vi "Measurement UI.vi"() -> ()   [LabVIEW 2025, in "Automotive Vision UI.lvlib"]
uses:
  Automotive Vision UI.lvlib
  <vilib>/vision/Image Controls.llb/IMAQ Image.ctl
  <vilib>/gRPC/LabVIEW gRPC Library/Shared/grpcId.ctl
  <vilib>/gRPC/LabVIEW gRPC Library/grpc-lvsupport-release.lvlib
  Automotive-Vision-OOBService_client/Automotive-Vision-OOBService_client.lvlib
  Automotive-Vision-OOBService_client/RPC Messages/hwval_ExportRequest.ctl
  Automotive-Vision-OOBService_client/RPC Messages/hwval_BoolRequest.ctl
  Automotive-Vision-OOBService_client/RPC Messages/hwval_ExportFileType.ctl
  Automotive-Vision-OOBService_client/RPC Messages/hwval_ExportTypeRequest.ctl
  auto vision config.ctl
  register.ctl
panel:
  out "COUNT LENGTH":u64
  out "REGISTERS":string[][](table)
  out "FRAME COUNT BYTES":u32[](array[numeric]) format="%02x"
  in  "config":string="{\n  \"RIO Device\":\"PXI1Slot4\",\n  \"Serial Channel\":\"SI0, SI1, SI2, SI3\",\n  \"SERDES Script\":\"C:\\\\dev\\\\ttashjia\\\\GSE\\\\Host\\\\Scripts\\\\DS90UB954\\\\Acq\\\\Loopback.py\",\n  \"POC Source\":0,\n  \"CSI-2 Data Source\":1,\n  \"Lane Count\":4,\n  \"Reference Clock\":25000000,\n  \"Image Data Type\":44,\n  \"Interpretation\":1,\n  \"Pattern\":3,\n  \"Algorithm\":0,\n  \"Virtual Channel\":0,\n  \"Embedded Data\":{\n    \"Pre-embedded Lines\":4,\n    \"Pre-embedded Line Length\":1920,\n    \"Post-embedded Lines\":2,\n    \"Post-embedded Line Length\":1920,\n    \"Frame Count\":{\"Line\":0,\"Offset\":2,\"Byte Count\":4}\n  },\n  \"Registers\":[\n    {\n      \"Name\":\"Temp0\",\n      \"Device\":97,\n      \"Address\":27,\n      \"Min\":0,\n      \"Max\":16\n    },\n    {\n      \"Name\":\"Temp1\",\n      \"Device\":97,\n      \"Address\":90,\n      \"Min\":0,\n      \"Max\":16\n    }\n  ],\n  \"Log Path\":\"C:\\\\data\"\n}"
  out "WIDTH":u64
  out "HEIGHT":u64
  out "Numeric":i32
  out "error out":errorcluster
  in  "GRPC status":string
  out "OOB gRPC Port":i32
  in  "BITFILE":string="IMAGE RESOLUTION: 800x600 - RAW12"
  out "Available SI Devices":string[][](array[string])
  in  "RIO HANDLER":string
  out "BYTES ACQUIRED":u64 format="%#.6p"
  out "ERROR":bool
  out "IMAGE PIXEL DATA":u32[](array[numeric])
  in  "IMAGE SAVE FORMAT":u32(ring) items=["PNG", "RAW LLP"]
  out "FRAME COUNT":u64
  out "IMAGE DATA":string
  in  "PAUSE":bool
  in  "CAPTURE":bool
  in  "PATH TO IMAGE CAPTURE":path=path "0"
  in  "SERIAL CHANNEL":string="SI1"
  out "SOURCE RATE (fps)":dbl
  out "STATE MESSAGE":string
  out "POC CURRENT (A)":dbl
  out "POC VOLTAGE (V)":dbl
  out "ACQ. DURATION (s)":dbl
  out "ACQ. IN PROGRESS":bool
  out "DISPLAY":T1(plugin-control)
  # "CONFIGURATION"
  # "Image path parameters"
  # "CONTROL"
  # "MONITOR"
  # "STATUS"
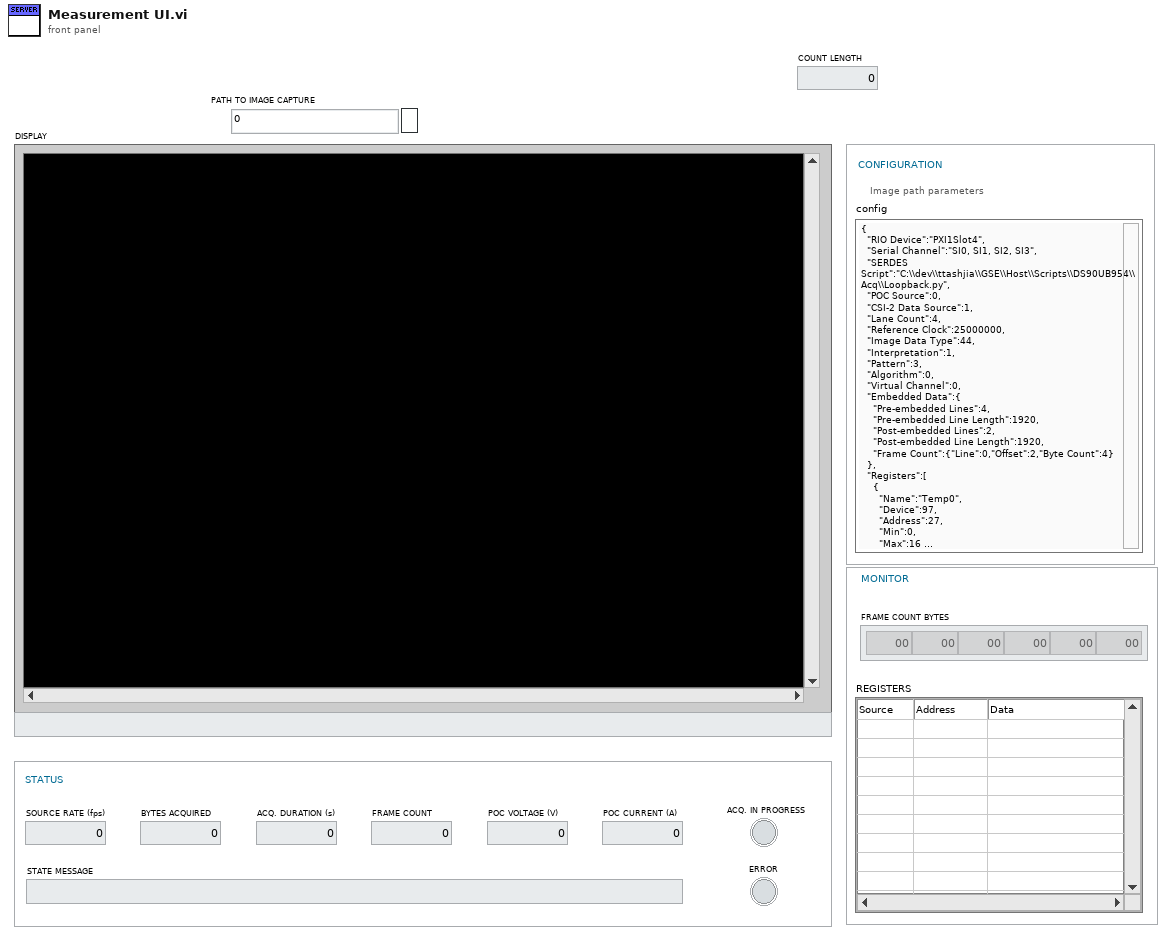
[diagram p1: front panel]
types:
  T1 = typedef "IMAQ Image.ctl" = refnum<image>
  T2 = typedef "Automotive Vision UI.lvlib/auto vision config.ctl" = cluster{"RIO Device":string, "Serial Channel":string, "SERDES Script":string, "POC Source":u32, "CSI-2 Data Source":u32, "Lane Count":u32, "Reference Clock":dbl, "Image Data Type":u32, "Interpretation":u32, "Pattern":u32, "Algorithm":u32, "Virtual Channel":u32, "Embedded Data":cluster{"Pre-embedded Lines":dbl, "Pre-embedded Line Length":dbl, "Post-embedded Lines":dbl, "Post-embedded Line Length":dbl, "Frame Count":cluster{"Line":dbl, "Offset":dbl, "Byte Count":dbl}}, "Registers":T3[], "Log Path":string}
  T3 = typedef "Automotive Vision UI.lvlib/register.ctl" = cluster{"Name":string, "Device":u8, "Address":u16, "Min":u16, "Max":u16}
  T4 = typedef "grpc-lvsupport-release.lvlib/grpcId.ctl" = u64
  T5 = cluster{"pattern":i32, "algorithm":i32, "red gain":dbl, "green gain":dbl, "blue gain":dbl}
  T6 = typedef "Automotive-Vision-OOBService_client.lvlib/hwval_BoolRequest.ctl" = cluster{"BooleanData":bool}
  T7 = typedef "Automotive-Vision-OOBService_client.lvlib/hwval_ExportRequest.ctl" = cluster{"FilePath":string}
  T8 = typedef "Automotive-Vision-OOBService_client.lvlib/hwval_ExportTypeRequest.ctl" = cluster{"FileType":T9}
  T9 = typedef "Automotive-Vision-OOBService_client.lvlib/hwval_ExportFileType.ctl" = enum32{"EXPORT_PNG", "EXPORT_RAW"}
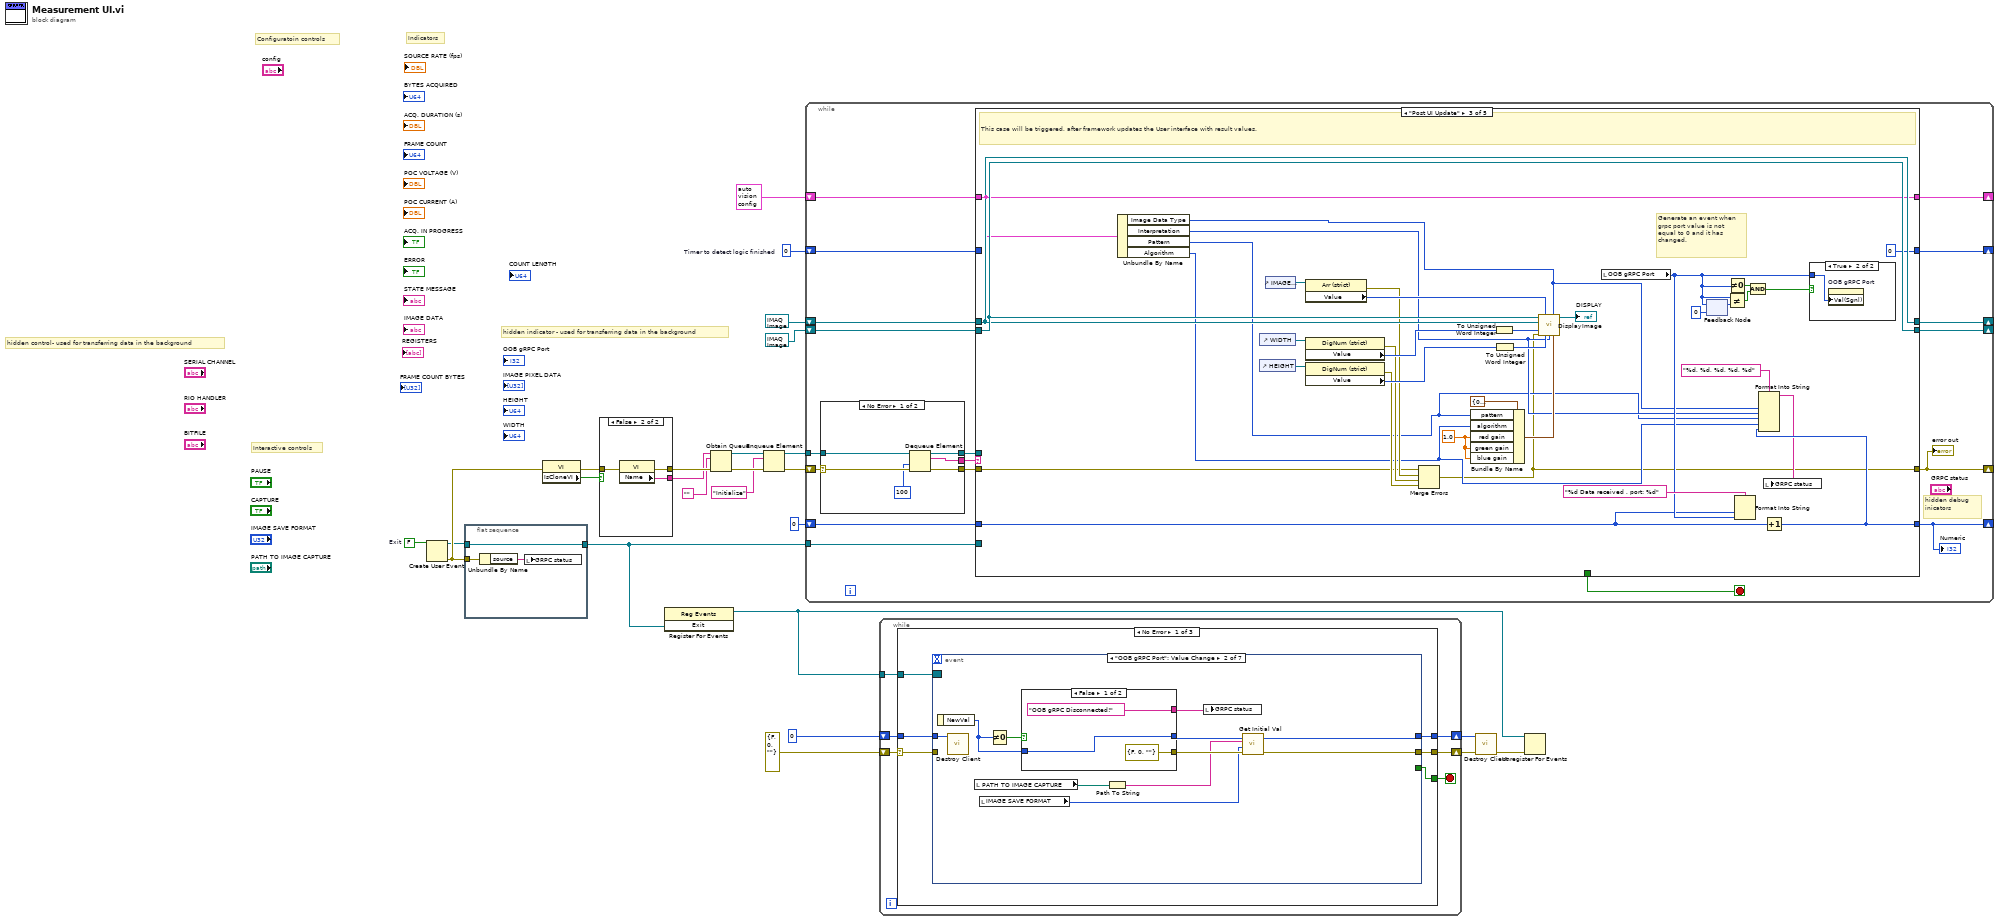
[diagram p0: block diagram]
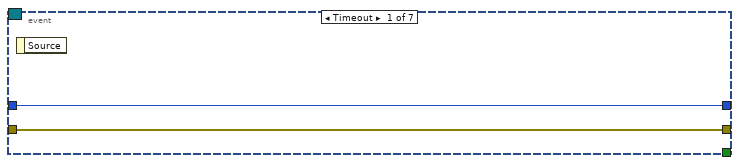
[diagram p2: hidden frame]
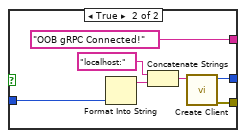
[diagram p3: hidden frame]
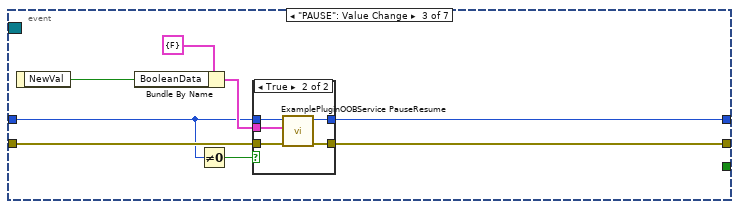
[diagram p4: hidden frame]
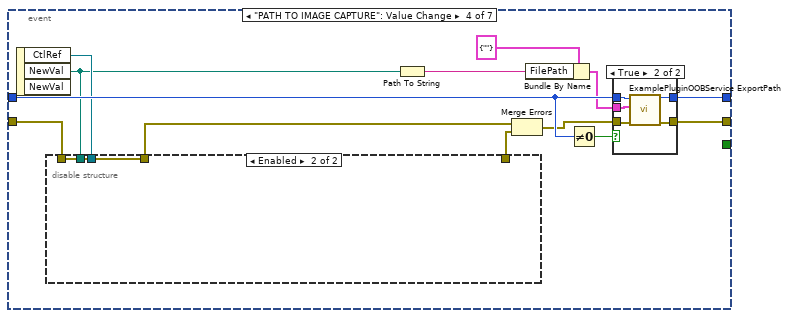
[diagram p6: hidden frame]
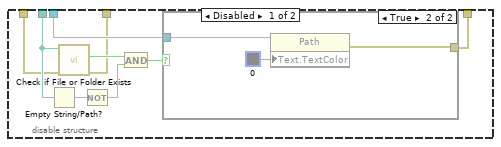
[diagram p7: hidden frame]
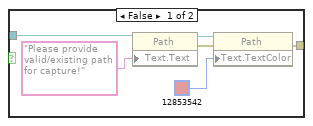
[diagram p8: hidden frame]
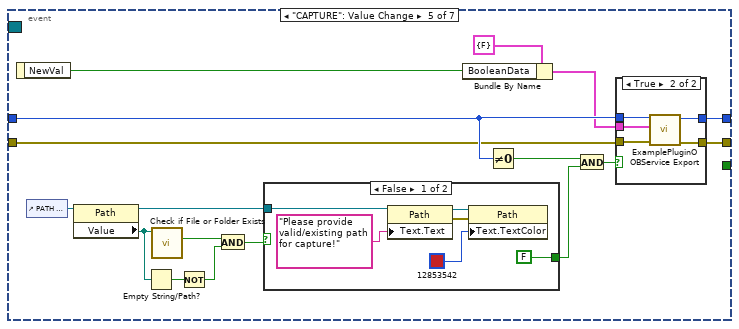
[diagram p10: hidden frame]
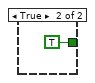
[diagram p11: hidden frame]
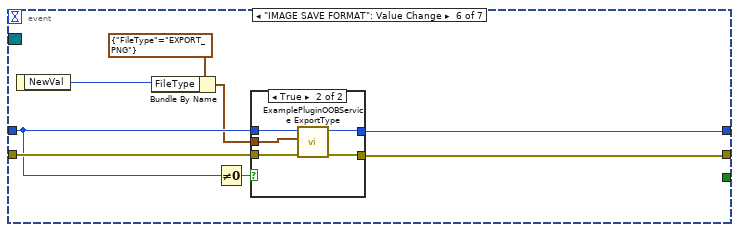
[diagram p13: hidden frame]
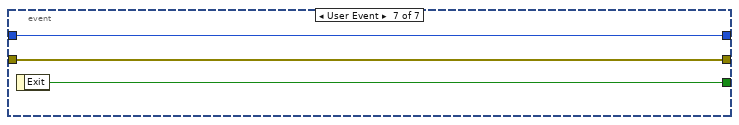
[diagram p15: hidden frame]
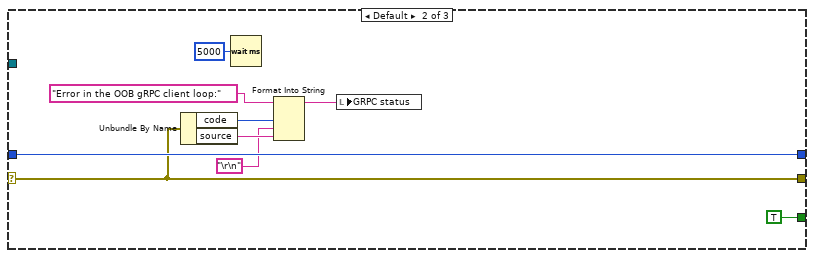
[diagram p16: hidden frame]
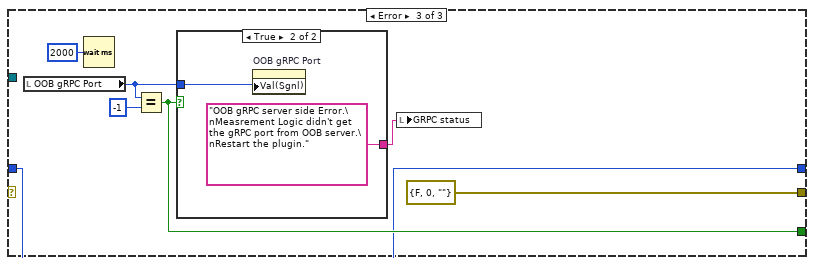
[diagram p17: hidden frame]
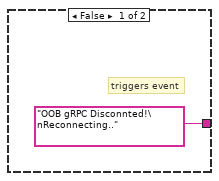
[diagram p18: hidden frame]
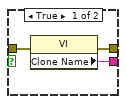
[diagram p19: hidden frame]
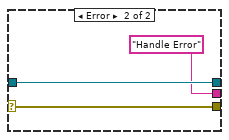
[diagram p20: hidden frame]
diagram:
  w6 = 0  # Timer to detect logic finished
  w15 = FALSE  # Exit
  # "Indicators"
  # "Configuratoin controls"
  # "Interactive controls"
  # "hidden indicator - used for transferring data in the background"
  # "hidden control- used for transferring data in the background"
  n1 = Create User Event(user event datatype=w15) -> (user event=w2:refnum<user-event>, error out=w8:errorcluster)  [unwired: 1 in]
  n2 = flat-sequence {
    tunnel: [w28] -> w9
    tunnel: w2 -> [w28]
    tunnel: w8 -> [w27]
    frame #0 {
      n3 = Unbundle By Name(w27) -> ("source"=w26:string)
      n4 = local write "GRPC status"(w26) -> ()
    }
  }
  n5 = property on="Property Node" class="VI"(error in=w8) -> (error out=w16:errorcluster, "IsCloneVI"=w17:bool)  [unwired: 1 in, 1 out]
  n6 = case shown="False" w17 {
    tunnel: [w31 w34] -> w25
    tunnel: [w30 w33] -> w24
    tunnel: w16 -> [w29 w32]
    frame True {
      n7 = property on="Property Node" class="VI"(error in=w29) -> (error out=w31:errorcluster, "Clone Name"=w30:string)  [unwired: 1 in, 1 out]
    }
    frame False {
      n8 = property on="Property Node" class="VI"(error in=w32) -> (error out=w34:errorcluster, "Name"=w33:string)  [unwired: 1 in, 1 out]
    }
  }
  n9 = register-events(w9) -> (reference out=w14:refnum<event-registration>)  [unwired: 2 in, 1 out]
  n10 = Obtain Queue(name (unnamed)=w24, element data type="" ("Empty String Constant"), error in (no error)=w25) -> (queue out=w21:refnum<queue>, error out=w23:errorcluster)  [unwired: 2 in, 1 out]
  n11 = Enqueue Element(queue=w21, element="Initialize", error in (no error)=w23) -> (queue out=w20:refnum<queue>, error out=w22:errorcluster)  [unwired: 1 in, 1 out]
  n12 = while {
    shift-right: [w41] -> _
    shift-left: w22 -> [w52]
    tunnel: w20 -> [w50]
    shift-right: [w43] -> _
    shift-left: T1 refnum ("Image Out Grayscale") -> [w45]
    shift-right: [w46] -> _
    shift-left: T1 refnum ("Image Out Grayscale") -> [w44]
    tunnel: w9 -> [w42]
    shift-right: [w39] -> _
    shift-left: 0 -> [w40]
    shift-right: [w37] -> _
    shift-left: w6 -> [w38]
    shift-right: [w35] -> _
    shift-left: T2 {"RIO Device"="", "Serial Channel"="", "SERDES Script"="", "POC Source"=0, "CSI-2 Data Source"=0, "Lane Count"=0, "Reference Clock"=0.0, "Image Data Type"=0, "Interpretation"=0, "Pattern"=0, "Algorithm"=0, "Virtual Channel"=0, "Embedded Data"={"Pre-embedded Lines"=0.0, "Pre-embedded Line Length"=0.0, "Post-embedded Lines"=0.0, "Post-embedded Line Length"=0.0, "Frame Count"={"Line"=0.0, "Offset"=0.0, "Byte Count"=0.0}}, "Registers"=[], "Log Path"=""} ("Auto Vision Config") -> [w36]
    stop <- w47 stop-if-true
    # "hidden debug inicators"
    n13 = case shown="No Error" w52 {
      selector: w52 -> [w58 w61]
      tunnel: [w57 w61] -> w51
      tunnel: w50 -> [w56 w60]
      tunnel: [w55 w60] -> w49
      tunnel: [w54 "Handle Error"] -> w48
      frame No Error {
        n14 = Dequeue Element(queue=w56, timeout in ms (-1)=100, error in (no error)=w58) -> (queue out=w55:refnum<queue>, element=w54:string, error out=w57:errorcluster)  [unwired: 1 out]
      }
      frame Error {
      }
    }
    n15 = case shown="\"Post UI Update\"" w48 {
      tunnel: w51 -> [w73 w143 w172 w208 w247]
      tunnel: w49 -> [w71 _ _ w231 w246]
      tunnel: [w74 w140 w162 w202 w245] -> w41
      tunnel: [_ FALSE _ TRUE TRUE] -> w47
      tunnel: [w62 w139 w196 w224 w252] -> w46
      tunnel: [w63 w138 w194 w224 w253] -> w43
      tunnel: w45 -> [w65 _ w194 w225 w253]
      tunnel: w44 -> [w64 _ w196 w226 w252]
      tunnel: w42 -> [_ _ _ w212 _]
      tunnel: w40 -> [_ _ w182 _ _]
      tunnel: [-3 1 w164 -1 -2] -> w39
      tunnel: [w68 0 ("Numeric 2") 0 ("Numeric 2") 0 ("Numeric 2") 0 ("Numeric 2")] -> w37
      tunnel: w38 -> [w69 _ _ _ _]
      tunnel: w36 -> [w67 w132 w170 w199 w242]
      tunnel: [w66 w141 w170 w199 w242] -> w35
      frame "Event", Default {
        n16 = event shown="[2] \"config\": Value Change" {
          selector: _ -> [_ _ _]
          dyn-events: _ -> [_ _ _]
          timeout: 100 -> [_ _ _]
          tunnel: [w78 w117 w123] -> w74
          tunnel: w73 -> [w81 w118 w129]
          tunnel: w71 -> [w80 w116 _]
          tunnel: w69 -> [w87 _ _]
          tunnel: [w86 _ _] -> w68
          tunnel: w67 -> [w77 w114 _]
          tunnel: [w77 w114 w124] -> w66
          tunnel: w65 -> [w75 w112 w130]
          tunnel: w64 -> [w76 w113 w128]
          tunnel: [w75 w112 w126] -> w63
          tunnel: [w76 w113 w125] -> w62
          event Timeout {
            n17 = event-data() -> ()  [unwired: 1 in, 3 out]
            n18 = control-ref of="ACQ. IN PROGRESS"() -> (w83:refnum<vi>)
            n19 = Increment(x=w87) -> (x+1=w86:i32)
            n20 = property on="Property Node" class="Bool (strict)"(reference=w83) -> ("Value"=w82:bool)  [unwired: 1 in, 2 out]
            n21 = Greater?(x=w86, y=10) -> (0:w84:bool)
            n22 = And(x=w84, y=w82) -> (x .and. y?=w79:bool)
            n23 = case shown="True" w79 {
              tunnel: w81 -> [w88 w90]
              tunnel: w80 -> [_ _]
              tunnel: [w88 w92] -> w78
              frame False {
              }
              frame True {
                # "Only update status to done if no error happend"
                n24 = control-ref of="ACQ. IN PROGRESS"() -> (w93:refnum<vi>)
                n25 = property on="Property Node" class="Bool (strict)"(reference=w93, error in=w90, "Value"=FALSE) -> (error out=w89:errorcluster)  [unwired: 1 out]
                n26 = control-ref of="STATE MESSAGE"() -> (w94:refnum<vi>)
                n27 = property on="Property Node" class="Str"(reference=w94, error in=w89) -> (reference out=w102:refnum<vi>, error out=w96:errorcluster, "Value"=w101:string)
                n28 = Search and Replace String(case sensitive?=TRUE ("ignore case? (F)"), input string=w101, search string="error", error in=w96) -> (number of replacements=w98:i32, error out=w95:errorcluster)  [unwired: 4 in, 2 out]
                n29 = Equal To 0?(x=w98) -> (x = 0?=w97:bool)
                n30 = case shown="True" w97 {
                  tunnel: w102 -> [_ w109]
                  tunnel: w101 -> [_ w107]
                  tunnel: w95 -> [w103 w105]
                  tunnel: [w103 w106] -> w92
                  frame False {
                  }
                  frame True {
                    n31 = Search and Replace String(input string=w107, search string="^.*", replace string="Done" ("replace string (\"\")"), error in=w105) -> (result string=w108:string, error out=w104:errorcluster)  [unwired: 4 in, 2 out]
                    n32 = property on="Property Node" class="Str"(reference=w109, error in=w104, "Value"=w108) -> (error out=w106:errorcluster)  [unwired: 1 out]
                  }
                }
              }
            }
          }
          event Panel Close? {
            n33 = event-data() -> ()  [unwired: 1 in, 4 out]
            n34 = Enqueue Element(queue=w116, element="Exit", error in (no error)=w118) -> (error out=w117:errorcluster)  [unwired: 1 in, 2 out]
            n35 = event-data ("Event Filter Node")("Discard?"=TRUE) -> ()  [unwired: 1 in, 1 out]
          }
          event "config": Value Change {
            n36 = event-data() -> ()  [unwired: 1 in, 6 out]
            n37 = call "IMAQ Dispose"("Image"=w130, "error in (no error)"=w129) -> ("error out"=w127:errorcluster)  [unwired: 4 in]
            n38 = property on="config" class="Str"() -> ("Value"=w120:string)  [unwired: 2 in, 2 out]
            n39 = call "IMAQ Dispose"("Image"=w128, "error in (no error)"=w127) -> ()  [unwired: 4 in, 1 out]
            n40 = Unflatten From JSON(JSON string=w120, type and defaults=T2 {"RIO Device"="", "Serial Channel"="", "SERDES Script"="", "POC Source"=0, "CSI-2 Data Source"=0, "Lane Count"=0, "Reference Clock"=0.0, "Image Data Type"=0, "Interpretation"=0, "Pattern"=0, "Algorithm"=0, "Virtual Channel"=0, "Embedded Data"={"Pre-embedded Lines"=0.0, "Pre-embedded Line Length"=0.0, "Post-embedded Lines"=0.0, "Post-embedded Line Length"=0.0, "Frame Count"={"Line"=0.0, "Offset"=0.0, "Byte Count"=0.0}}, "Registers"=[], "Log Path"=""} ("Auto Vision Config")) -> (value=w124:T2)  [unwired: 5 in, 1 out]
            n41 = Unbundle By Name(w124) -> ("Serial Channel"=w121:string, "Image Data Type"=w122:u32)
            n42 = call "InitImageDisplay.vi"("payload data type"=w122, "SI channel"=w121) -> ("error out"=w123:errorcluster, "Image Out Color"=w125:T1, "Image Out Grayscale"=w126:T1)  [unwired: 7 in]
          }
        }
      }
      frame "Initialize" {
        (unwired) 0
        # "Do a default selection for SI0"
        # "select SI cha."
        # "select 0. device in list"
        # "used to store device data between events"
        n43 = property on="config" class="Str"(error in=w143) -> (error out=w142:errorcluster, "Value"=w133:string)  [unwired: 1 in, 1 out]
        n44 = Empty String/Path?(string/path=w133) -> (empty?=w134:bool)
        n45 = case shown="False" w134 {
          tunnel: w133 -> [w159 _]
          tunnel: w142 -> [w158 _]
          tunnel: [w156 w160] -> w141
          tunnel: [w155 44] -> w136
          tunnel: w132 -> [_ w160]
          frame False {
            n46 = Unflatten From JSON(JSON string=w159, type and defaults=T2 {"RIO Device"="", "Serial Channel"="", "SERDES Script"="", "POC Source"=0, "CSI-2 Data Source"=0, "Lane Count"=0, "Reference Clock"=0.0, "Image Data Type"=0, "Interpretation"=0, "Pattern"=0, "Algorithm"=0, "Virtual Channel"=0, "Embedded Data"={"Pre-embedded Lines"=0.0, "Pre-embedded Line Length"=0.0, "Post-embedded Lines"=0.0, "Post-embedded Line Length"=0.0, "Frame Count"={"Line"=0.0, "Offset"=0.0, "Byte Count"=0.0}}, "Registers"=[], "Log Path"=""} ("Auto Vision Config"), error in (no error)=w158) -> (value=w156:T2)  [unwired: 4 in, 1 out]
            n47 = Unbundle By Name(w156) -> ("Image Data Type"=w155:u32)
          }
          frame True {
          }
        }
        n48 = call "GetChimeraResources.vi"("error in (no error)"=w143) -> ("error out"=w137:errorcluster, "Available input channels on Automotive Camera Vision Devices"=w152:string[][])  [unwired: 7 in, 2 out]
        "Available SI Devices" <- w152
        n49 = Index Array(array=w152) -> (element=w148:string[])  [unwired: 2 in]
        n50 = Array Subset(array=w148, index=2) -> (w151:string[])  [unwired: 1 in]
        n51 = Index Array(array=w148, index #1=0 ("index"), index #2=1 ("index")) -> (element #1=w149:string, element #2=w145:string)
        n52 = Index Array(array=w151) -> (element=w135:string)  [unwired: 1 in]
        n53 = local write "RIO HANDLER"(w149) -> ()
        n54 = local write "BITFILE"(w145) -> ()
        n55 = local write "SERIAL CHANNEL"(w135) -> ()
        n56 = call "InitImageDisplay.vi"("error in (no error)"=w137, "payload data type"=w136, "SI channel"=w135) -> ("error out"=w140:errorcluster, "Image Out Color"=w139:T1, "Image Out Grayscale"=w138:T1)  [unwired: 6 in]
      }
      frame "Post UI Update" {
        w191 = 1.0 ("red gain")
        # "Generate an event when grpc port value is not equal to 0 and it has changed."
        # "This case will be triggered, after framework updates the User interface with result values."
        n57 = Unbundle By Name(w170) -> ("Image Data Type"=w168:u32, "Interpretation"=w167:u32, "Pattern"=w166:u32, "Algorithm"=w165:u32)
        n58 = control-ref of="WIDTH"() -> (w181:refnum<vi>)
        n59 = control-ref of="HEIGHT"() -> (w180:refnum<vi>)
        n60 = control-ref of="IMAGE PIXEL DATA"() -> (w197:refnum<vi>)
        n61 = property on="Property Node" class="Arr (strict)"(reference=w197) -> (error out=w175:errorcluster, "Value"=w193:u32[])  [unwired: 1 in, 1 out]
        n62 = property on="Property Node" class="DigNum (strict)"(reference=w181) -> (error out=w174:errorcluster, "Value"=w179:u64)  [unwired: 1 in, 1 out]
        n63 = property on="Property Node" class="DigNum (strict)"(reference=w180) -> (error out=w173:errorcluster, "Value"=w177:u64)  [unwired: 1 in, 1 out]
        n64 = Merge Errors(w172, w175, w174, w173) -> (w162:errorcluster)
        n65 = Bundle By Name(cluster=T5 {"pattern"=0, "algorithm"=0, "red gain"=0.0, "green gain"=0.0, "blue gain"=0.0} ("bayer parameters"), "pattern"=w166, "algorithm"=w165, "red gain"=w191, "green gain"=w191, "blue gain"=w191) -> (w190:T5)
        n66 = To Unsigned Word Integer(number=w179) -> (unsigned 16bit integer=w178:u16)
        n67 = To Unsigned Word Integer(number=w177) -> (unsigned 16bit integer=w176:u16)
        n68 = call "DisplayImage.vi"("image color"=w196, "Image Pixel Data"=w193, "data type"=w168, "Image grayscale"=w194, "width"=w178, "error in (no error)"=w162, "height"=w176, "interpretation"=w167, "bayer parameters"=w190) -> ("display image"=→"DISPLAY":T1)  [unwired: 5 in, 1 out]
        n69 = local read "OOB gRPC Port"() -> (w183:i32)
        n70 = feedback #1(0 ("OOB gRPC Port")) -> (w186:i32)
        n71 = feedback-in #1(w183) -> ()
        n72 = Not Equal?(x=w183, y=w186) -> (x != y?=w187:bool)
        n73 = Not Equal To 0?(x=w183) -> (x != 0?=w188:bool)
        n74 = Format Into String(format string="%d Data received , port: %d" ("GRPC status"), w182, w183) -> ()  [unwired: 2 in, 2 out]
        n75 = Compound Arithmetic op=AND(w188, w187) -> (w185:bool)
        n76 = Increment(x=w182) -> (x+1=w164:i32)
        n77 = Format Into String(format string="%d, %d, %d, %d, %d" ("GRPC status"), w168, w167, w166, w165, w164) -> (resulting string=w163:string)  [unwired: 2 in, 1 out]
        n78 = local write "GRPC status"(w163) -> ()
        n79 = case shown="True" w185 {
          tunnel: w183 -> [_ w198]
          frame False {
          }
          frame True {
            n80 = property on="OOB gRPC Port" class="DigNum (strict)"("Val(Sgnl)"=w198) -> ()  [unwired: 2 in, 2 out]
          }
        }
      }
      frame "Exit" {
        w224 = T1 refnum ("Image Out Grayscale")
        # "Only update status to done if no error happend"
        # "This case is triggered to close the User Interface from framework"
        n81 = call "IMAQ Dispose"("Image"=w226) -> ("error out"=w227:errorcluster)  [unwired: 5 in]
        n82 = Flush Queue(queue=w231, error in (no error)=w208) -> (queue out=w230:refnum<queue>, error out=w229:errorcluster)  [unwired: 1 out]
        n83 = Generate User Event(user event=w212, event data cluster=TRUE ("event data")) -> (user event out=w213:refnum<user-event>, error out=w200:errorcluster)  [unwired: 2 in]
        n84 = call "IMAQ Dispose"("Image"=w225, "error in (no error)"=w227) -> ("error out"=w207:errorcluster)  [unwired: 4 in]
        n85 = Release Queue(queue=w230, force destroy? (F)=TRUE, error in (no error)=w229) -> (error out=w211:errorcluster)  [unwired: 2 out]
        n86 = Destroy User Event(user event=w213, error in=w200) -> (error out=w210:errorcluster)
        n87 = Merge Errors(w207, w211, w210) -> (w206:errorcluster)
        n88 = control-ref of="ACQ. IN PROGRESS"() -> (w223:refnum<vi>)
        n89 = property on="Property Node" class="Bool (strict)"(reference=w223, error in=w206, "Value"=FALSE) -> (error out=w205:errorcluster)  [unwired: 1 out]
        n90 = control-ref of="STATE MESSAGE"() -> (w221:refnum<vi>)
        n91 = property on="Property Node" class="Str"(reference=w221, error in=w205) -> (reference out=w220:refnum<vi>, error out=w204:errorcluster, "Value"=w219:string)
        n92 = Search and Replace String(case sensitive?=TRUE ("ignore case? (F)"), input string=w219, search string="error", error in=w204) -> (number of replacements=w216:i32, error out=w203:errorcluster)  [unwired: 4 in, 2 out]
        n93 = Equal To 0?(x=w216) -> (x = 0?=w215:bool)
        n94 = case shown="False" w215 {
          tunnel: w220 -> [_ w239]
          tunnel: w219 -> [_ w237]
          tunnel: w203 -> [w233 w235]
          tunnel: [w233 w236] -> w202
          frame False {
          }
          frame True {
            n95 = Search and Replace String(input string=w237, search string="^.*", replace string="Done" ("replace string (\"\")"), error in=w235) -> (result string=w238:string, error out=w234:errorcluster)  [unwired: 4 in, 2 out]
            n96 = property on="Property Node" class="Str"(reference=w239, error in=w234, "Value"=w238) -> (error out=w236:errorcluster)  [unwired: 1 out]
          }
        }
      }
      frame "Handle Error" {
        n97 = Flush Queue(queue=w246, error in (no error)=w247) -> (queue out=w250:refnum<queue>, error out=w249:errorcluster)  [unwired: 1 out]
        n98 = Release Queue(queue=w250, force destroy? (F)=TRUE, error in (no error)=w249) -> (error out=w245:errorcluster)  [unwired: 2 out]
      }
    }
    "error out" <- w41
    "Numeric" <- w39
  }
  n99 = while {
    tunnel: w14 -> [w256]
    shift-right: [w257] -> w12
    shift-left: errorcluster {"status"=FALSE, "code"=0, "source"=""} ("error IO") -> [w259]
    shift-right: [w254] -> w10
    shift-left: T4 0 ("gRPC ID out") -> [w255]
    stop <- w258 stop-if-true
    n100 = case shown="No Error" w259 {
      selector: w259 -> [w263 w393 _]
      tunnel: [w260 TRUE w405] -> w258
      tunnel: [w264 w393 errorcluster {"status"=FALSE, "code"=0, "source"=""} ("error IO")] -> w257
      tunnel: w256 -> [w265 _ _]
      tunnel: w255 -> [w262 w398 w403]
      tunnel: [w261 w398 w403] -> w254
      frame No Error {
        n101 = event shown="[1] \"OOB gRPC Port\": Value Change" {
          selector: w265 -> [_ _ _ _ _ _ _]
          dyn-events: _ -> [_ _ _ _ _ _ _]
          timeout: _ -> [_ _ _ _ _ _ _]
          tunnel: [w267 w272 w294 w314 w358 w378 w388] -> w264
          tunnel: w263 -> [w267 _ w293 w303 w351 w379 w388]
          tunnel: w262 -> [w266 w274 w289 w312 w357 w377 w389]
          tunnel: [w266 w271 w295 w315 w356 w376 w389] -> w261
          tunnel: [_ _ _ _ _ _ w390] -> w260
          event Timeout {
            n102 = event-data() -> ()  [unwired: 1 in, 1 out]
          }
          event "OOB gRPC Port": Value Change {
            n103 = event-data() -> ("NewVal"=w275:i32)  [unwired: 1 in]
            n104 = call "Destroy Client.vi"("gRPC ID"=w274) -> ()  [unwired: 10 in, 1 out]
            n105 = local read "PATH TO IMAGE CAPTURE"() -> (w269:path)
            n106 = local read "IMAGE SAVE FORMAT"() -> (w270:u32)
            n107 = Not Equal To 0?(x=w275) -> (x != 0?=w276:bool)
            n108 = case shown="False" w276 {
              tunnel: [errorcluster {"status"=FALSE, "code"=0, "source"=""} ("error out") w281] -> w277
              tunnel: w275 -> [w280 w285]
              tunnel: [w280 w282] -> w271
              tunnel: ["OOB gRPC Disconnected!" ("Status") "OOB gRPC Connected!" ("Status")] -> w273
              frame False {
              }
              frame True {
                n109 = Format Into String(w285) -> (resulting string=w287:string)  [unwired: 3 in, 1 out]
                n110 = Concatenate Strings("localhost:" ("string"), w287) -> (w283:string)
                n111 = call "Create Client.vi"("address"=w283) -> ("error out"=w281:errorcluster, "gRPC ID Out"=w282:T4)  [unwired: 9 in]
              }
            }
            n112 = Path To String(path=w269) -> (string=w268:string)
            n113 = local write "GRPC status"(w273) -> ()
            n114 = call "Get Initial Val.vi"("error in"=w277, "IMAGE SAVE FORMAT"=w270, "String"=w268, "gRPC ID In"=w271) -> ("error out"=w272:errorcluster)  [unwired: 7 in]
          }
          event "PAUSE": Value Change {
            n115 = event-data() -> ("NewVal"=w291:bool)  [unwired: 1 in]
            n116 = Bundle By Name(cluster=T6 {"BooleanData"=FALSE} ("Request Data"), "BooleanData"=w291) -> (w292:T6)
            n117 = Not Equal To 0?(x=w289) -> (x != 0?=w290:bool)
            n118 = case shown="True" w290 {
              tunnel: [w297 w301] -> w295
              tunnel: [w296 w300] -> w294
              tunnel: w289 -> [w297 w302]
              tunnel: w293 -> [w296 w299]
              tunnel: w292 -> [_ w298]
              frame False {
              }
              frame True {
                n119 = call "ExamplePluginOOBService PauseResume.vi"("error in"=w299, "Request Data"=w298, "gRPC ID"=w302) -> ("error out"=w300:errorcluster, "gRPC ID out"=w301:T4)  [unwired: 6 in, 1 out]
              }
            }
          }
          event "PATH TO IMAGE CAPTURE": Value Change {
            n120 = event-data() -> ("CtlRef"=w308:refnum<vi>, "NewVal"=w307:path)  [unwired: 1 in, 1 out]
            n121 = disable-structure shown="Enabled" {
              disable-tunnel: w308 -> [w324 _]
              disable-tunnel: w307 -> [w320 _]
              disable-tunnel: [w318 _] -> w305
              disable-tunnel: [w317 w334] -> w304
              disable-tunnel: w303 -> [w316 w334]
              frame Disabled {
                n122 = Empty String/Path?(string/path=w320) -> (empty?=w323:bool)
                n123 = call <vilib>:"Check if File or Folder Exists.vi"("error in (no error)"=w316, "path"=w320) -> ("error out"=w317:errorcluster, "file or folder exists?"=w322:bool)  [unwired: 7 in, 1 out]
                n124 = Not(x=w323) -> (.not. x?=w321:bool)
                n125 = And(x=w322, y=w321) -> (x .and. y?=w319:bool)
                n126 = case shown="True" w319 {
                  tunnel: w324 -> [w330 w333]
                  tunnel: [w325 w331] -> w318
                  frame False {
                    n127 = property on="Property Node" class="Path"(reference=w330, "Text.Text"="Please provide valid/existing path for capture!" ("Path Text.Text")) -> (reference out=w329:refnum<vi>, error out=w328:errorcluster)  [unwired: 1 in]
                    n128 = property on="Property Node" class="Path"(reference=w329, error in=w328, "Text.TextColor"=u32 12853542 ("Path Text.Text Colors:Text Color")) -> (error out=w325:errorcluster)  [unwired: 1 out]
                  }
                  frame True {
                    n129 = property on="Property Node" class="Path"(reference=w333, "Text.TextColor"=u32 0 ("Path Text.Text Colors:Text Color")) -> (error out=w331:errorcluster)  [unwired: 1 in, 1 out]
                  }
                }
              }
              frame Enabled {
              }
            }
            n130 = Path To String(path=w307) -> (string=w310:string)
            n131 = Merge Errors(w304, w305) -> (w306:errorcluster)
            n132 = Bundle By Name(cluster=T7 {"FilePath"=""} ("Request Data"), "FilePath"=w310) -> (w309:T7)
            n133 = Not Equal To 0?(x=w312) -> (x != 0?=w313:bool)
            n134 = case shown="True" w313 {
              tunnel: [w336 w340] -> w315
              tunnel: [w335 w338] -> w314
              tunnel: w312 -> [w336 w341]
              tunnel: w306 -> [w335 w339]
              tunnel: w309 -> [_ w337]
              frame False {
              }
              frame True {
                n135 = call "ExamplePluginOOBService ExportPath.vi"("error in"=w339, "Request Data"=w337, "gRPC ID"=w341) -> ("error out"=w338:errorcluster, "gRPC ID out"=w340:T4)  [unwired: 6 in, 1 out]
              }
            }
          }
          event "CAPTURE": Value Change {
            n136 = event-data() -> ("NewVal"=w354:bool)  [unwired: 1 in]
            n137 = control-ref of="PATH TO IMAGE CAPTURE"() -> (w347:refnum<vi>)
            n138 = property on="Property Node" class="Path"(reference=w347) -> (reference out=w352:refnum<vi>, "Value"=w346:path)  [unwired: 1 in, 1 out]
            n139 = Empty String/Path?(string/path=w346) -> (empty?=w345:bool)
            n140 = call <vilib>:"Check if File or Folder Exists.vi"("path"=w346) -> ("file or folder exists?"=w343:bool)  [unwired: 8 in, 2 out]
            n141 = Not(x=w345) -> (.not. x?=w342:bool)
            n142 = And(x=w343, y=w342) -> (x .and. y?=w344:bool)
            n143 = case shown="False" w344 {
              tunnel: w352 -> [w364 _]
              tunnel: [FALSE TRUE] -> w348
              frame False {
                n144 = property on="Property Node" class="Path"(reference=w364, "Text.Text"="Please provide valid/existing path for capture!" ("Path Text.Text")) -> (reference out=w363:refnum<vi>, error out=w362:errorcluster)  [unwired: 1 in]
                n145 = property on="Property Node" class="Path"(reference=w363, error in=w362, "Text.TextColor"=u32 12853542 ("Path Text.Text Colors:Text Color")) -> ()  [unwired: 2 out]
              }
              frame True {
              }
            }
            n146 = Bundle By Name(cluster=T6 {"BooleanData"=FALSE} ("Request Data"), "BooleanData"=w354) -> (w353:T6)
            n147 = Not Equal To 0?(x=w357) -> (x != 0?=w350:bool)
            n148 = And(x=w350, y=w348) -> (x .and. y?=w349:bool)
            n149 = case shown="True" w349 {
              tunnel: w351 -> [w366 w372]
              tunnel: [w366 w371] -> w358
              tunnel: w357 -> [w367 w370]
              tunnel: [w367 w369] -> w356
              tunnel: w353 -> [_ w368]
              frame False {
              }
              frame True {
                n150 = call "ExamplePluginOOBService Export.vi"("error in"=w372, "Request Data"=w368, "gRPC ID"=w370) -> ("error out"=w371:errorcluster, "gRPC ID out"=w369:T4)  [unwired: 6 in, 1 out]
              }
            }
          }
          event "IMAGE SAVE FORMAT": Value Change {
            n151 = event-data() -> ("NewVal"=w374:u32)  [unwired: 1 in]
            n152 = Bundle By Name(cluster=T8 {"FileType"=enum."EXPORT_PNG"} ("Request Data"), "FileType"=w374) -> (w373:T8)
            n153 = Not Equal To 0?(x=w377) -> (x != 0?=w380:bool)
            n154 = case shown="True" w380 {
              tunnel: w379 -> [w381 w385]
              tunnel: [w381 w384] -> w378
              tunnel: w377 -> [w382 w386]
              tunnel: [w382 w383] -> w376
              tunnel: w373 -> [_ w387]
              frame False {
              }
              frame True {
                n155 = call "ExamplePluginOOBService ExportType.vi"("error in"=w385, "Request Data"=w387, "gRPC ID"=w386) -> ("error out"=w384:errorcluster, "gRPC ID out"=w383:T4)  [unwired: 6 in, 1 out]
              }
            }
          }
          event User Event {
            n156 = event-data() -> ("Exit"=w390:bool)  [unwired: 1 in]
          }
        }
      }
      frame Default {
        n157 = Unbundle By Name(w393) -> ("code"=w397:i32, "source"=w396:string)
        n158 = Wait (ms)(milliseconds to wait=u32 5000) -> ()  [unwired: 1 out]
        n159 = Format Into String(initial string="Error in the OOB gRPC client loop:" ("format string"), w397, "\r\n" ("End of Line Constant"), w396) -> (resulting string=w391:string)  [unwired: 2 in, 1 out]
        n160 = local write "GRPC status"(w391) -> ()
      }
      frame Error {
        n161 = local read "OOB gRPC Port"() -> (w401:i32)
        n162 = Wait (ms)(milliseconds to wait=u32 2000) -> ()  [unwired: 1 out]
        n163 = Equal?(x=w401, y=-1 ("x")) -> (x = y?=w405:bool)
        n164 = case shown="True" w405 {
          tunnel: ["OOB gRPC Disconnted!\nReconnecting.." ("Status") "OOB gRPC server side Error.\nMeasrement Logic didn't get the gRPC port from OOB server.\nRestart the plugin." ("Status")] -> w400
          tunnel: w401 -> [_ w408]
          frame False {
            # "triggers event"
          }
          frame True {
            n165 = property on="OOB gRPC Port" class="DigNum (strict)"("Val(Sgnl)"=w408) -> ()  [unwired: 2 in, 2 out]
          }
        }
        n166 = local write "GRPC status"(w400) -> ()
      }
    }
  }
  n167 = call "Destroy Client.vi"("error in"=w12, "gRPC ID"=w10) -> ("error out"=w11:errorcluster)  [unwired: 9 in]
  n168 = Unregister For Events(event registration refnum=w14, error in=w11) -> ()  [unwired: 1 out]
